vi "JKI State Machine Helper - VI Tree.vi"   [LabVIEW 2020]
uses:
  JKI State Machine API/source/JKI SM/JKI SM.lvclass
  <vilib>/Utility/miscctls.llb/LVPositionTypeDef.ctl
  PopupMenu Plugin/JKI SM Helper.llb/JKI SM Helper Source.ctl
  JKI State Machine API/source/Support/State Call Cluster.ctl
  JKI State Machine API/source/Support/State Calls Array.ctl
types:
  T1 = typedef "State Calls Array.ctl" = T2[]
  T2 = typedef "State Call Cluster.ctl" = cluster{"StringConstant":refnum<vi>, "Structure":string, "Frame Name":string, "State Call":string}
  T3 = typedef "JKI SM Helper Source.ctl" = cluster{"Case Structure":refnum<vi>[], "Event Structure":refnum<vi>[], "While Loop":refnum<vi>[], "String Constant":refnum<vi>[], "Named Bundler":refnum<vi>[], "Named Unbundler":refnum<vi>[], "InPlaceClusterNode":refnum<vi>[], "Wire":refnum<vi>[]}
  T4 = typedef "LVPositionTypeDef.ctl" = cluster{"Left":i32, "Top":i32}
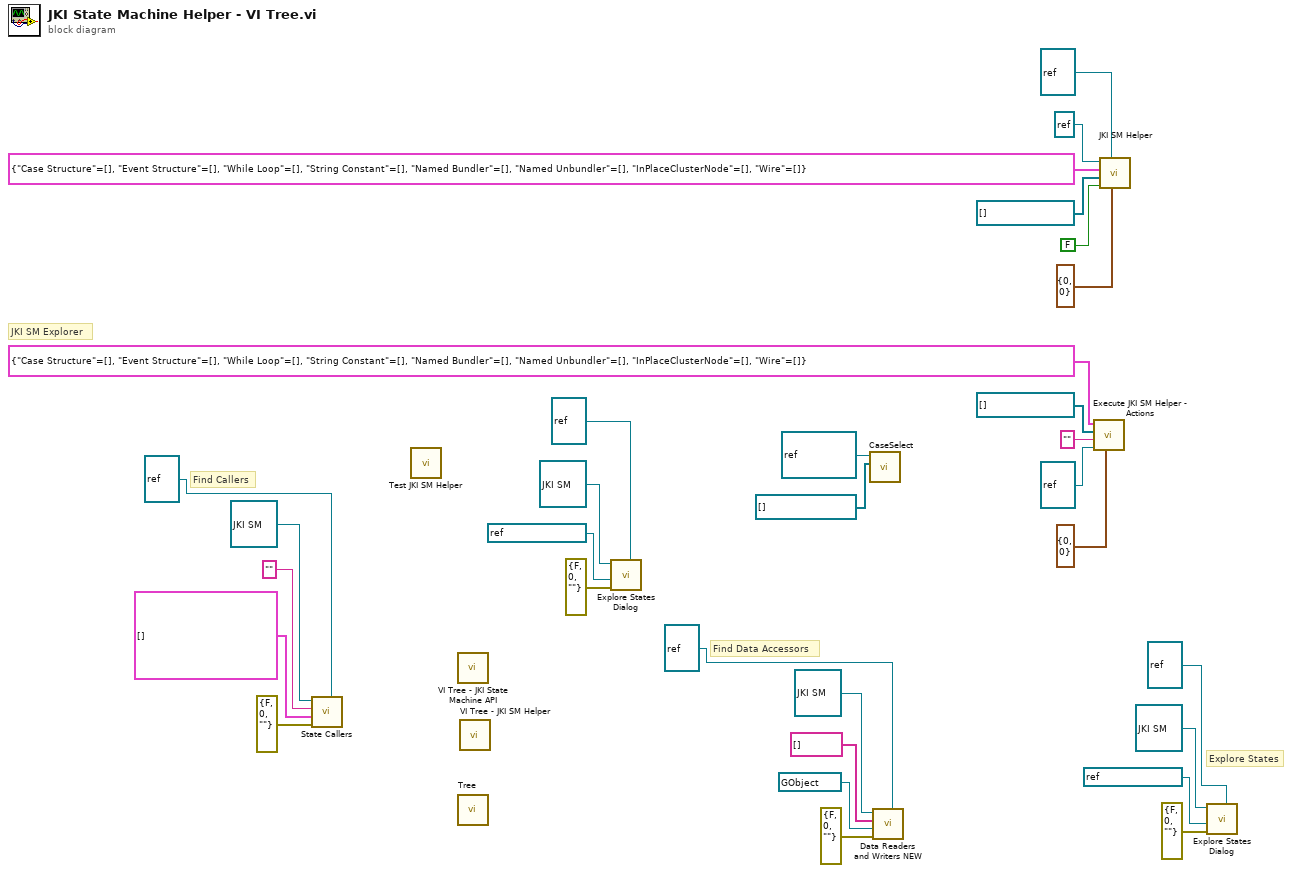
[diagram p0: block diagram]
diagram:
  # "Explore States"
  # "Find Callers"
  # "Find Data Accessors"
  # "JKI SM Explorer"
  n1 = call "State Callers.vi"("Calling VI Ref"=refnum<vi> refnum, "error in (no error)"=errorcluster {"status"=FALSE, "code"=0, "source"=""}, "Callers"=T1 [], "State"="", "JKI SM in"=refnum<class "JKI SM.lvclass"> refnum) -> ()  [unwired: 6 in, 1 out]
  n2 = call "Test JKI SM Helper.vi"() -> ()  [unwired: 12 in]
  n3 = call "VI Tree - JKI State Machine API.vi"() -> ()  [unwired: 12 in]
  n4 = call "Tree.vi"() -> ()  [unwired: 1 in]
  n5 = call "VI Tree - JKI SM Helper.vi"() -> ()  [unwired: 12 in]
  n6 = call "Explore States Dialog.vi"("Calling VI Ref"=refnum<vi> refnum, "error in (no error)"=errorcluster {"status"=FALSE, "code"=0, "source"=""}, "StringConstant"=refnum<vi> refnum, "JKI SM in"=refnum<class "JKI SM.lvclass"> refnum) -> ()  [unwired: 7 in, 1 out]
  n7 = call "CaseSelect.vi"("SelList[]"=refnum<vi>[] [], "Startup Callback"=refnum<notifier> refnum) -> ()  [unwired: 10 in]
  n8 = call "Data Readers and Writers NEW.vi"("Calling VI Ref"=refnum<vi> refnum, "error in (no error)"=errorcluster {"status"=FALSE, "code"=0, "source"=""}, "(Un)Bundler"=refnum<vi> refnum, "Full Element Name"=string[] [], "JKI SM in"=refnum<class "JKI SM.lvclass"> refnum) -> ()  [unwired: 6 in, 1 out]
  n9 = call "Execute JKI SM Helper - Actions.vi"("Mouse Position"=T4 {"Left"=0, "Top"=0}, "User VI Ref"=refnum<vi> refnum, "Menu Item Tag Suffix"="", "Remaining Items"=refnum<vi>[] [], "Affected Items"=T3 {"Case Structure"=[], "Event Structure"=[], "While Loop"=[], "String Constant"=[], "Named Bundler"=[], "Named Unbundler"=[], "InPlaceClusterNode"=[], "Wire"=[]}) -> ()  [unwired: 6 in, 1 out]
  n10 = call "JKI SM Helper.vi"("Mouse Position"=T4 {"Left"=0, "Top"=0}, "User VI Ref"=refnum<vi> refnum, "Is Multi-select?"=FALSE, "Remaining Items"=refnum<vi>[] [], "Affected Items"=T3 {"Case Structure"=[], "Event Structure"=[], "While Loop"=[], "String Constant"=[], "Named Bundler"=[], "Named Unbundler"=[], "InPlaceClusterNode"=[], "Wire"=[]}, "Menu Refnum"=refnum<k9> refnum) -> ()  [unwired: 5 in, 1 out]
  n11 = call "Explore States Dialog.vi"("Calling VI Ref"=refnum<vi> refnum, "error in (no error)"=errorcluster {"status"=FALSE, "code"=0, "source"=""}, "StringConstant"=refnum<vi> refnum, "JKI SM in"=refnum<class "JKI SM.lvclass"> refnum) -> ()  [unwired: 7 in, 1 out]
